vi "Search-computer.vi"(8 "error in (no error)":errorcluster caption="错误输入（无错误）", 11 "Ignote coefficient 输入":refnum<class "Coefficient.lvclass">) -> (0 "error out":errorcluster caption="错误输出", 2 "数值":i32, 3 "Ignote coefficient 输出":refnum<class "Coefficient.lvclass">)   [LabVIEW 2025, in "Coefficient.lvclass"]
uses:
  Coefficient.lvclass
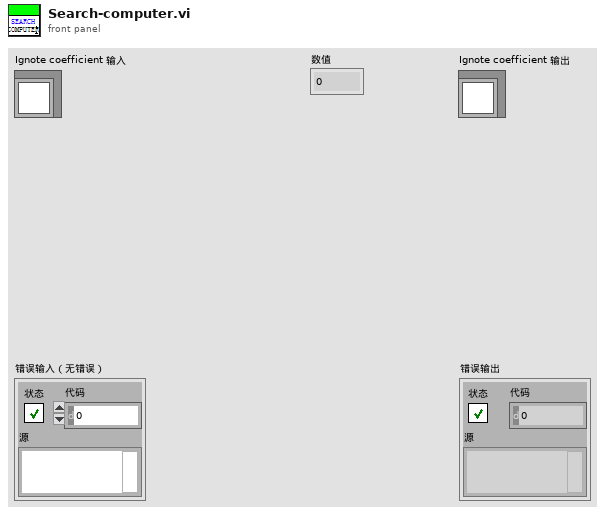
[diagram p1: front panel]
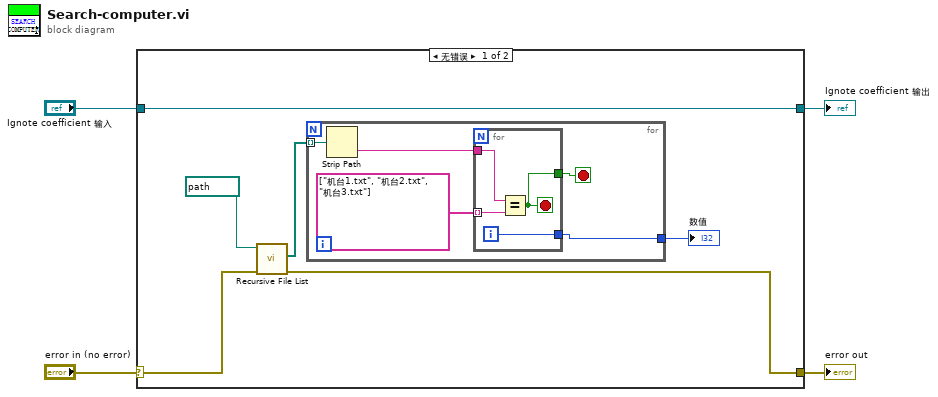
[diagram p0: block diagram]
diagram:
  n1 = case shown="无错误" "error in (no error)" {
    selector: "error in (no error)" -> [w8 w21]
    tunnel: [w7 w21] -> w3
    tunnel: [w10 w20] -> w1
    tunnel: "Ignote coefficient 输入" -> [w10 w20]
    frame No Error {
      n2 = call <vilib>:"Recursive File List.vi"("error in (no error)"=w8, "Folder Path"=path "C:/机台" ("stripped path")) -> ("error out"=w7:errorcluster, "All Files in Dir"=w6:path[])  [unwired: 5 in, 3 out]
      n3 = for {
        tunnel: w6 -> [w13] mode=indexing
        tunnel: [w11] -> w5
        stop <- w12 stop-if-true
        n4 = Strip Path(path=w13) -> (name=w14:string)  [unwired: 1 out]
        n5 = for {
          tunnel: string[] ["机台1.txt", "机台2.txt", "机台3.txt"] ("正则表达式") -> [w19] mode=indexing
          tunnel: w14 -> [w18]
          tunnel: [w17] -> w12
          tunnel: [w16] -> w11
          i -> [w16]
          stop <- w17 stop-if-true
          n6 = Equal?(x=w18, y=w19) -> (x = y?=w17:bool)
        }
      }
      "数值" <- w5
    }
    frame Error {
    }
  }
  "error out" <- w3
  "Ignote coefficient 输出" <- w1
